vi "sample obtain bucket put object.vi"() -> ()   [LabVIEW 2015]
uses:
  GET Object Result Parameters.ctl
  Core/HTTP Request/AWS Credentials.ctl
  PUT Object Request Parameters.ctl
  ACL.ctl
  Storage Class.ctl
  Core/HTTP Request/Name Value Pair.ctl
  GET Object Request Parameters.ctl
  Core/Request Range.ctl
  Bucket/Bucket.lvclass
  Core/HTTP Request/HTTP Request.lvclass
  NI_AWS_S3.lvlib
  Core/NI_AWS_Core.lvlib
panel:
  out "object key":string
  out "GetObjectResult":T1
  out "Object Data":string
  out "error out":errorcluster
  in  "Bucket name":string="bpreis-test-96"
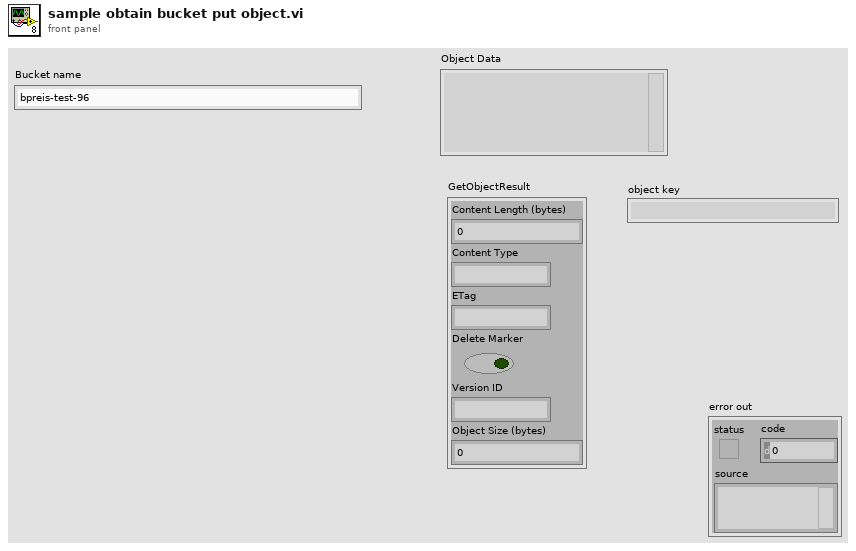
[diagram p1: front panel]
types:
  T1 = typedef "NI_AWS_S3.lvlib/GET Object Result Parameters.ctl" = cluster{"Content Length (bytes)":u64, "Content Type":string, "ETag":string, "Delete Marker":bool, "Version ID":string, "Object Size (bytes)":u64}
  T2 = typedef "NI_AWS_S3.lvlib/GET Object Request Parameters.ctl" = cluster{"Range":T3, "If Modified Since":timestamp, "If Unmodified Since":timestamp, "Matching ETag":string, "Nonmatching ETag":string}
  T3 = typedef "NI_AWS_Core.lvlib/Request Range.ctl" = cluster{"Start":i64, "Length":i64}
  T4 = typedef "NI_AWS_S3.lvlib/PUT Object Request Parameters.ctl" = cluster{"Content Type":string, "ACL":T5, "Storage Class":T6, "User-Defined Metadata":T7[]}
  T5 = typedef "NI_AWS_S3.lvlib/ACL.ctl" = enum16{"private", "public-read", "public-read-write", "aws-exec-read", "authenticated-read", "bucket-owner-read", "bucket-owner-full-control"}
  T6 = typedef "NI_AWS_S3.lvlib/Storage Class.ctl" = enum16{"STANDARD", "REDUCED_REDUNDANCY"}
  T7 = typedef "NI_AWS_Core.lvlib/HTTP Request.lvclass/Name Value Pair.ctl" = cluster{"name":string, "value":string}
  T8 = typedef "NI_AWS_Core.lvlib/HTTP Request.lvclass/AWS Credentials.ctl" = cluster{"Access Key":string, "Secret Key":string}
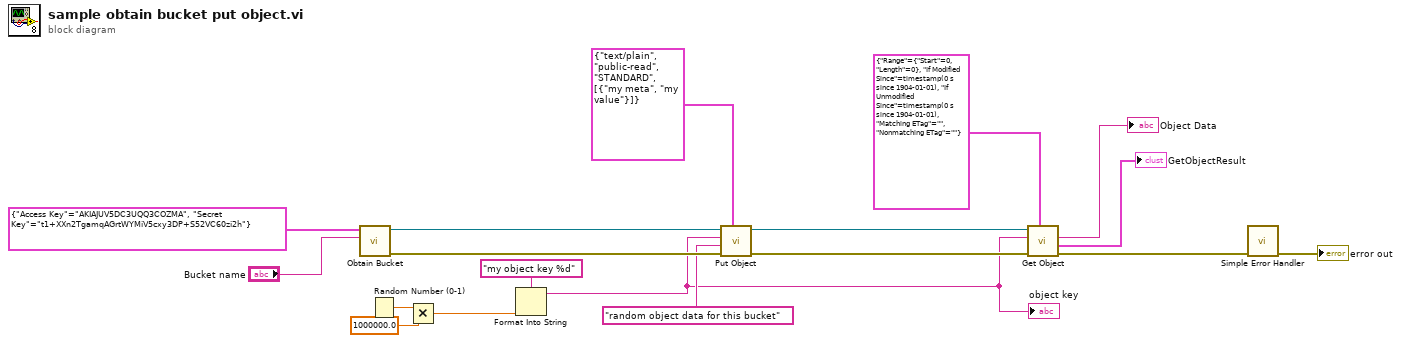
[diagram p0: block diagram]
diagram:
  n1 = call "Obtain Bucket.vi"("Bucket name"="Bucket name", "AWS Credentials"=T8 {"Access Key"="AKIAJUV5DC3UQQ3COZMA", "Secret Key"="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"}) -> ("error out"=w18:errorcluster, "Bucket"=w14:refnum<class "Bucket.lvclass">)  [unwired: 8 in]
  n2 = Random Number (0-1)() -> (number: 0 to 1=w4:dbl)
  n3 = Multiply(x=w4, y=1000000.0) -> (x*y=w2:dbl)
  n4 = Format Into String(format string="my object key %d" ("Object Key"), w2) -> (resulting string=w5:string)  [unwired: 2 in, 1 out]
  "object key" <- w5
  n5 = call "Put Object.vi"("Object Parameters"=T4 {"Content Type"="text/plain", "ACL"=enum."public-read", "Storage Class"=enum."STANDARD", "User-Defined Metadata"=[{"name"="my meta", "value"="my value"}]} ("PUT Object Request Parameters"), "error in (no error)"=w18, "Object Data"="random object data for this bucket", "Object Path"=w5, "Bucket in"=w14) -> ("error out"=w11:errorcluster, "Bucket out"=w9:refnum<class "Bucket.lvclass">)  [unwired: 5 in]
  n6 = call "Get Object.vi"("Request Parameters"=T2 {"Range"={"Start"=0, "Length"=0}, "If Modified Since"=timestamp(0 s since 1904-01-01), "If Unmodified Since"=timestamp(0 s since 1904-01-01), "Matching ETag"="", "Nonmatching ETag"=""}, "error in (no error)"=w11, "Object Path"=w5, "Bucket in"=w9) -> ("error out"=w10:errorcluster, "Object Info"=→"GetObjectResult":T1, "Data"=→"Object Data":string)  [unwired: 3 in, 2 out]
  n7 = call <vilib>:"Simple Error Handler.vi"("error in (no error)"=w10) -> ("error out"=→"error out":errorcluster)  [unwired: 4 in, 4 out]
